vi "Get VI Name.vi"(11 "VI Call In":refnum<class "VI Call.lvclass">) -> (2 "VI Name":string)   [LabVIEW 2020, in "VI Call.lvclass"]
uses:
  VI Call.lvclass
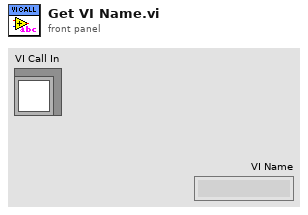
[diagram p1: front panel]
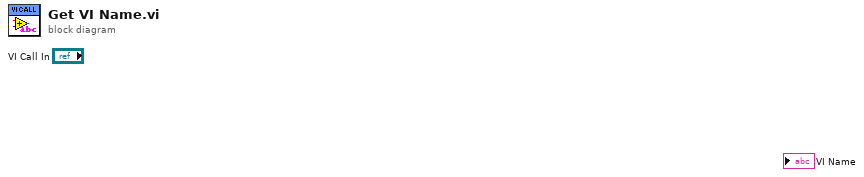
[diagram p0: block diagram]
diagram:
